vi "Send TX Message.vi"(8 "error in (no error)":errorcluster, 10 "element":string, 11 "RxTx in":refnum<class "RxTx.lvclass">) -> (0 "error out":errorcluster, 3 "RxTx out":refnum<class "RxTx.lvclass">)   [LabVIEW 2018, in "RxTx.lvclass"]
uses:
  RxTx.lvclass
  RxTx.lvclass/RxTx.ctl
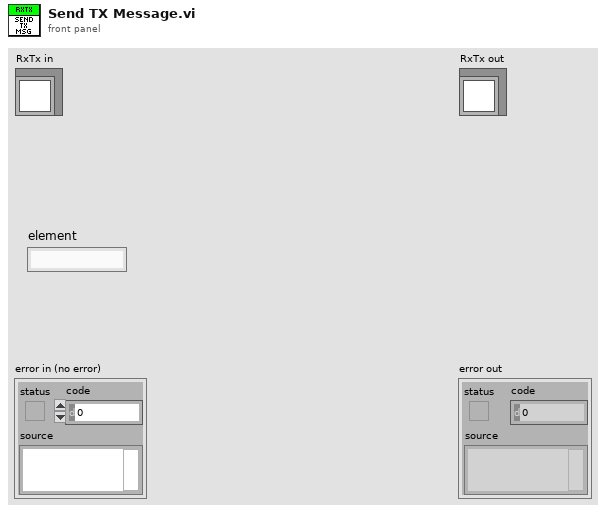
[diagram p1: front panel]
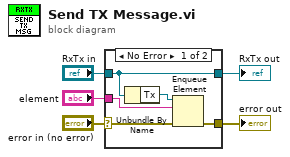
[diagram p0: block diagram]
diagram:
  n1 = case shown="No Error" "error in (no error)" {
    selector: "error in (no error)" -> [w9 w12]
    tunnel: [w6 w12] -> w4
    tunnel: [w8 w11] -> w2
    tunnel: "RxTx in" -> [w8 w11]
    tunnel: "element" -> [w7 _]
    frame No Error {
      n2 = Unbundle By Name(w8) -> ("Tx"=w10:refnum<queue>)
      n3 = Enqueue Element(queue=w10, element=w7, error in (no error)=w9) -> (error out=w6:errorcluster)  [unwired: 1 in, 2 out]
    }
    frame Error {
    }
  }
  "error out" <- w4
  "RxTx out" <- w2
